vi "Create Lib if not Present.vi"(7 "plug-in name":string, 8 "error in":errorcluster, 9 "dest directory":path, 10 "project ref":refnum<vi>, 11 "virtual folder ref":refnum<vi>) -> (0 "error out":errorcluster, 3 "library refnum":refnum<vi>)   [LabVIEW 2021, in "Multiple Converter.lvlib"]
uses:
  Multiple Converter.lvlib
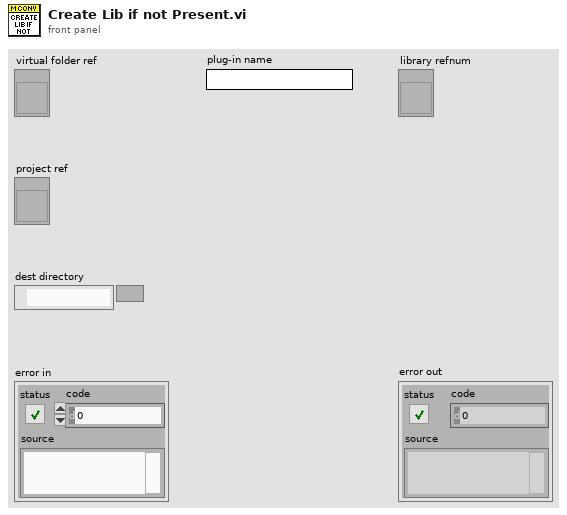
[diagram p1: front panel]
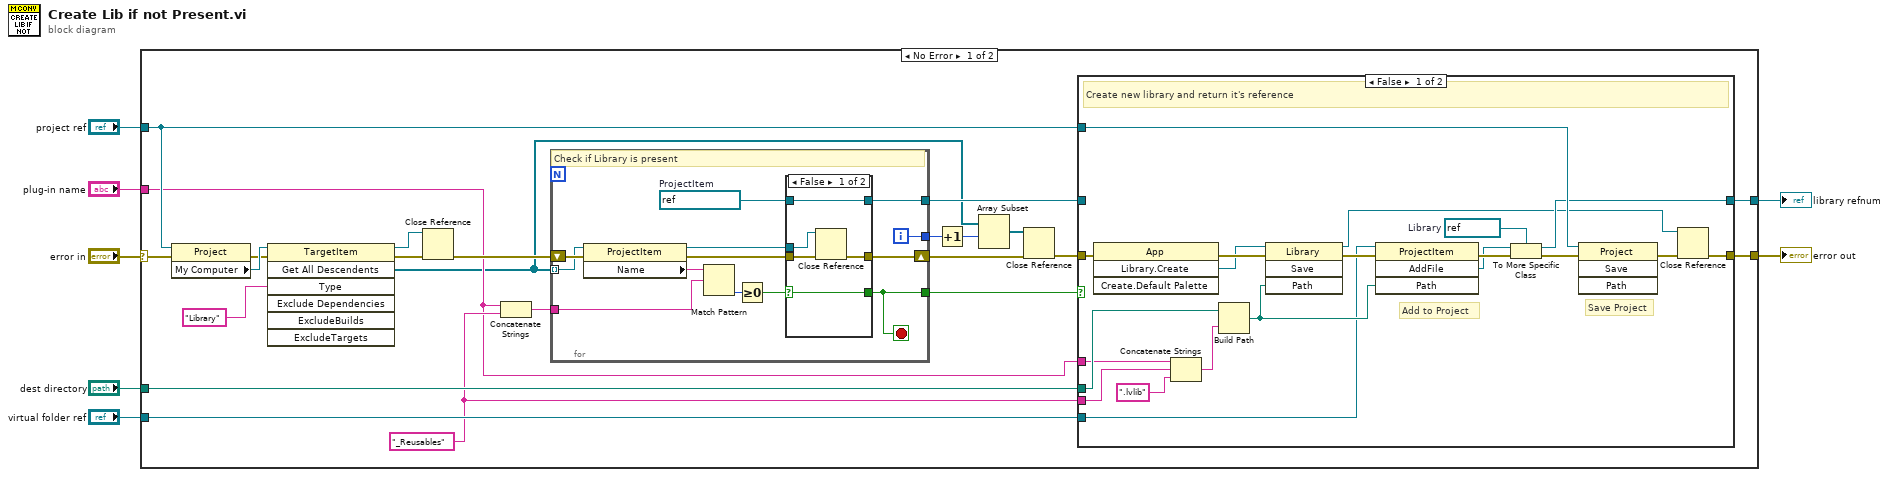
[diagram p0: block diagram]
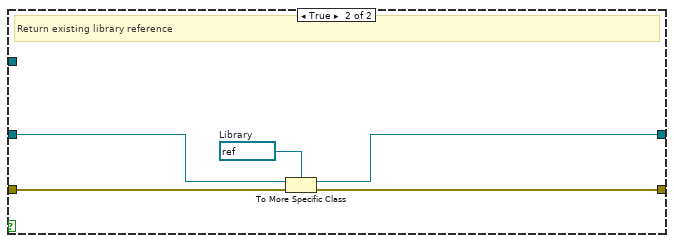
[diagram p2: hidden frame]
diagram:
  n1 = case shown="No Error" "error in" {
    selector: "error in" -> [w22 w77]
    tunnel: "dest directory" -> [w21 _]
    tunnel: "virtual folder ref" -> [w20 _]
    tunnel: "project ref" -> [w19 _]
    tunnel: [w18 w77] -> w3
    tunnel: [w16 _] -> w2
    tunnel: "plug-in name" -> [w14 _]
    frame No Error {
      w15 = "_Reusables" ("string")
      n2 = property class="Project"(reference=w19, error in=w22) -> (error out=w26:errorcluster, "My Computer"=w30:refnum<vi>)  [unwired: 1 out]
      n3 = invoke class="TargetItem" method="Get All Descendents"(reference=w30, error in=w26, "Type"="Library") -> (reference out=w27:refnum<vi>, error out=w28:errorcluster, "All Descendents"=w12:refnum<vi>[])  [unwired: 4 in, 4 out]
      n4 = Close Reference(reference=w27, error in (no error)=w28) -> (error out=w25:errorcluster)
      n5 = Concatenate Strings(w14, w15) -> (w24:string)
      n6 = for {
        tunnel: w12 -> [w67] mode=indexing
        tunnel: [w60] -> w17
        tunnel: w24 -> [w59]
        tunnel: [w57] -> w23
        tunnel: [w58] -> w10
        shift-right: [w56] -> w8
        shift-left: w25 -> [w68]
        i -> [w58]
        stop <- w57 stop-if-true
        w63 = refnum<vi> refnum  # ProjectItem
        # "Check if Library is present"
        n7 = property class="ProjectItem"(reference=w67, error in=w68) -> (reference out=w62:refnum<vi>, error out=w61:errorcluster, "Name"=w66:string)
        n8 = Match Pattern(string=w66, regular expression=w59) -> (offset past match=w65:i32)  [unwired: 1 in, 3 out]
        n9 = Greater Or Equal To 0?(x=w65) -> (x >= 0?=w64:bool)
        n10 = case shown="False" w64 {
          selector: w64 -> [w70 w75]
          tunnel: w62 -> [w71 w76]
          tunnel: [w73 w74] -> w56
          tunnel: [w72 w76] -> w60
          tunnel: w63 -> [w72 _]
          tunnel: [w70 w75] -> w57
          tunnel: w61 -> [w69 w74]
          frame False {
            n11 = Close Reference(reference=w71, error in (no error)=w69) -> (error out=w73:errorcluster)
          }
          frame True {
          }
        }
      }
      n12 = Increment(x=w10) -> (x+1=w9:i32)
      n13 = Array Subset(array=w12, index=w9) -> (w11:refnum<vi>[])  [unwired: 1 in]
      n14 = Close Reference(reference=w11, error in (no error)=w8) -> (error out=w13:errorcluster)
      n15 = case shown="False" w23 {
        tunnel: w13 -> [w50 w55]
        tunnel: w21 -> [w48 _]
        tunnel: w20 -> [w42 _]
        tunnel: w19 -> [w41 _]
        tunnel: [w35 w54] -> w18
        tunnel: w17 -> [_ w52]
        tunnel: [w36 w53] -> w16
        tunnel: w15 -> [w32 _]
        tunnel: w14 -> [w31 _]
        frame False {
          w37 = refnum<vi> refnum  # Library
          # "Save Project"
          # "Add to Project"
          # "Create new library and return it's reference"
          n16 = invoke class="App" method="Library.Create"(error in=w50) -> (error out=w49:errorcluster, "Create Library"=w46:refnum<vi>)  [unwired: 3 in, 2 out]
          n17 = Concatenate Strings(w31, w32, ".lvlib" ("string")) -> (w47:string)
          n18 = Build Path(base path=w48, name or relative path=w47) -> (appended path=w43:path)
          n19 = invoke class="Library" method="Save"(reference=w46, error in=w49, "Path"=w43) -> (reference out=w34:refnum<vi>, error out=w44:errorcluster)  [unwired: 1 in, 2 out]
          n20 = invoke class="ProjectItem" method="AddFile"(reference=w42, error in=w44, "Path"=w43) -> (error out=w45:errorcluster, "AddFile"=w38:refnum<vi>)  [unwired: 1 in, 2 out]
          n21 = To More Specific Class(target class=w37, reference=w38, error in=w45) -> (specific class reference=w36:refnum<vi>, error out=w39:errorcluster)
          n22 = invoke class="Project" method="Save"(reference=w41, error in=w39) -> (error out=w40:errorcluster)  [unwired: 2 in, 3 out]
          n23 = Close Reference(reference=w34, error in (no error)=w40) -> (error out=w35:errorcluster)
        }
        frame True {
          w51 = refnum<vi> refnum  # Library
          # "Return existing library reference"
          n24 = To More Specific Class(target class=w51, reference=w52, error in=w55) -> (specific class reference=w53:refnum<vi>, error out=w54:errorcluster)
        }
      }
    }
    frame Error {
    }
  }
  "error out" <- w3
  "library refnum" <- w2
